vi "RT_IO_Acquisition_Loop.vi"(8 "error in (no error)":errorcluster={"status"=FALSE, "code"=0, "source"="\"\""}, 10 "sample policy":string, 11 "NI hardware references":string) -> (0 "error out":errorcluster={"status"=FALSE, "code"=0, "source"="\"\""}, 2 "status ok":bool, 3 "Typed process value updates":string)   [LabVIEW 2026]
doc: "INTENT: Read sensor channels with quality/timestamps. LOGIC: Read configured analog/digital channels, scale/calibrate, timestamp and publish bounded snapshots."
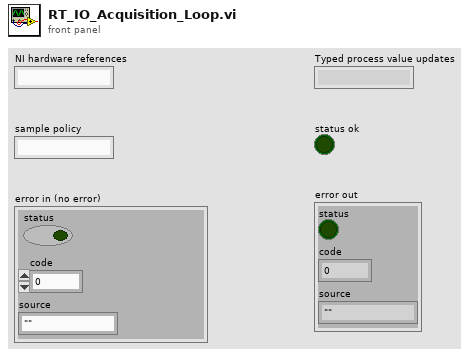
[diagram p1: front panel]
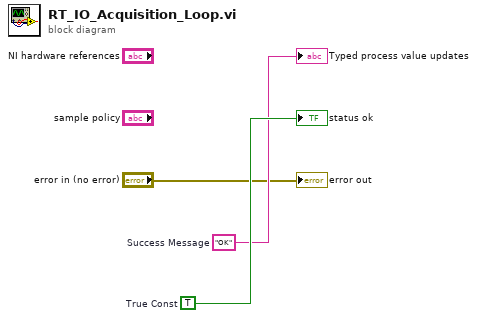
[diagram p0: block diagram]
diagram:
  w3 = TRUE  # True Const
  w2 = "OK"  # Success Message
  "Typed process value updates" <- w2
  "status ok" <- w3
  "error out" <- "error in (no error)"
